vi "Maximum Interval.vi"() -> (0 "Maximum interval (ms)":u32)   [LabVIEW 2021, in "Interval Timer.lvlib"]
doc: "Return the longest-possible interval in milliseconds."
uses:
  Interval Timer.lvlib
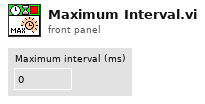
[diagram p1: front panel]
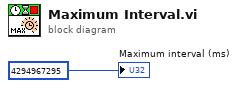
[diagram p0: block diagram]
diagram:
  "Maximum interval (ms)" <- u32 4294967295 ("New Acquisition Time")
